vi "Native_DeleteGObject.vi"() -> ()   [LabVIEW 2024]
panel:
  out "error out":errorcluster caption="错误输出"
  in  "object_id":u32
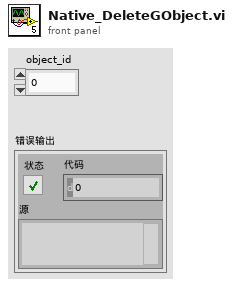
[diagram p1: front panel]
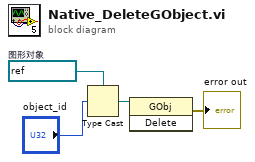
[diagram p0: block diagram]
diagram:
  w3 = refnum<vi> refnum  # 图形对象
  n1 = Type Cast ("强制类型转换")(type=w3, x="object_id") -> (*(type *) &x=w2:refnum<vi>)
  n2 = invoke class="GObj" method="Delete"(reference=w2) -> (error out=→"error out":errorcluster)  [unwired: 2 in, 2 out]
